vi "FuncVI-dtstr.vi"(5 "InstanceRef":T2, 9 "arg list":T1[](array[typedef]) {"num" format="%.2f"}) -> (0 "error out":bool, 3 "result":T1 {"num" format="%.2f"})   [LabVIEW 2021]
doc: "::: CalcExpress Toolkit :::\nCopyright (c) 2000-2026 Konstantin Shifershteyn. All rights reserved."
uses:
  cetypes.llb/CalcExpress Function Argument Info.ctl
  cetypes.llb/CalcExpress Instance RefNum.ctl
panel:
  in  "max arg num":i32=2
  in  "min arg num":i32
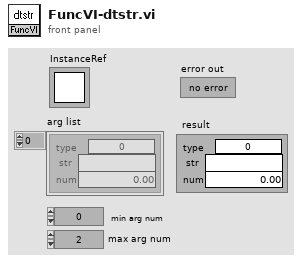
[diagram p1: front panel]
types:
  T1 = typedef "CalcExpress Function Argument Info.ctl" = cluster{"type":u32, "str":string, "num":dbl}
  T2 = typedef "CalcExpress Instance RefNum.ctl" = refnum<k1>
  T3 = cluster{"index":i32, "data type":enum32{"String", "DBL Number", "identifier", "1D Array of DBL", "2D Array of DBL", "CDB Number", "1D Array of CDB", "2D Array of CDB", "1D Array of String", "2D Array of String", "Unknown data type"}, "default num":dbl, "default str":string}
  T4 = cluster{"index":i32, "any type":i32, "default num":dbl, "default str":string}
  T5 = cluster{"index":i32, "any type":u32, "default num":dbl, "default str":string}[]
  T6 = enum32{"String", "DBL Number", "identifier", "1D Array of DBL", "2D Array of DBL", "CDB Number", "1D Array of CDB", "2D Array of CDB", "1D Array of String", "2D Array of String", "Unknown data type"}
  T7 = cluster{"data type":enum32{"String", "DBL Number", "identifier", "1D Array of DBL", "2D Array of DBL", "CDB Number", "1D Array of CDB", "2D Array of CDB", "1D Array of String", "2D Array of String", "Unknown data type"}, "data string":string, "num":dbl}
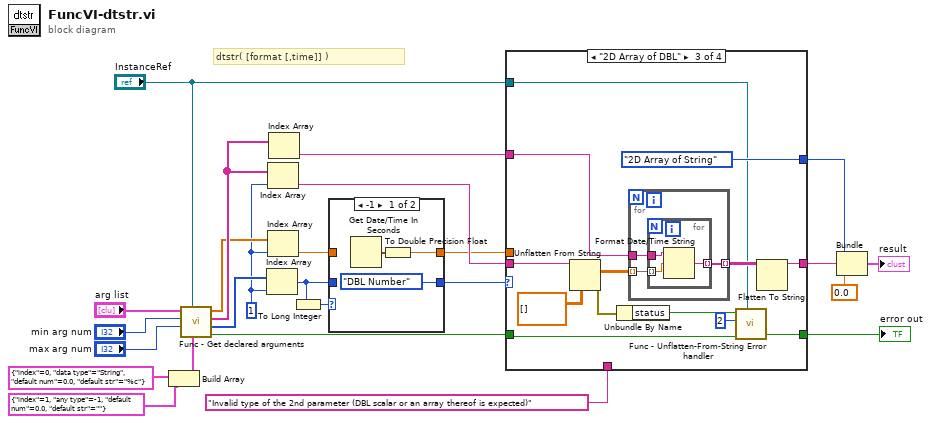
[diagram p0: block diagram]
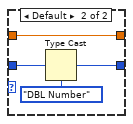
[diagram p2: hidden frame]
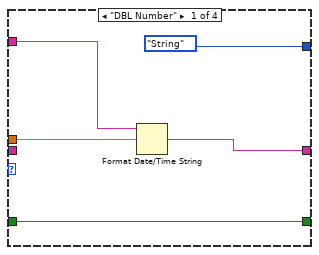
[diagram p3: hidden frame]
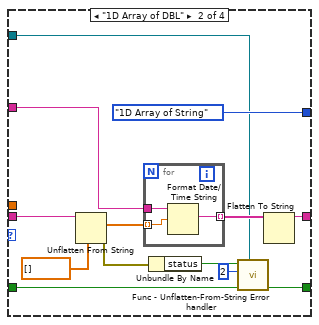
[diagram p4: hidden frame]
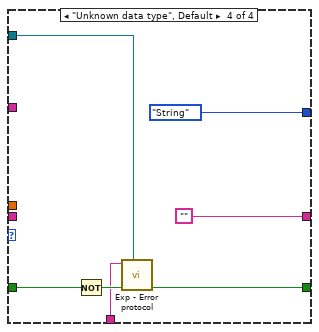
[diagram p5: hidden frame]
diagram:
  w6 = 1
  # "dtstr( [format [,time]] )"
  n1 = Build Array(T3 {"index"=0, "data type"=enum."String", "default num"=0.0, "default str"="%c"} ("arg descriptor"), T4 {"index"=1, "any type"=-1, "default num"=0.0, "default str"=""} ("arg descriptor")) -> (w23:T5)
  n2 = call "Func - Get declared arguments.vi"("arg descriptors"=w23, "InstanceRef"="InstanceRef", "max arg num"="max arg num", "min arg num"="min arg num", "arg list"="arg list") -> ("error out"=w19:bool, "type list"=w20:u32[], "str list"=w15:string[], "num list"=w14:dbl[])  [unwired: 3 in]
  n3 = Index Array(array=w20, index=w6) -> (element=w9:u32)
  n4 = Index Array(array=w15, index=w6) -> (element=w24:string)
  n5 = Index Array(array=w14, index=w6) -> (element=w7:dbl)
  n6 = Index Array(array=w15) -> (element=w21:string)  [unwired: 1 in]
  n7 = To Long Integer(number=w9) -> (32bit integer=w5:i32)
  n8 = case shown="-1" w5 {
    tunnel: [T6."DBL Number" ("data type") w30] -> w22
    tunnel: w9 -> [_ w31]
    tunnel: [w28 w32] -> w8
    tunnel: w7 -> [_ w32]
    frame -1 {
      n9 = Get Date/Time In Seconds() -> (seconds since 1Jan1904=w27:timestamp)
      n10 = To Double Precision Float(number=w27) -> (double precision float=w28:dbl)
    }
    frame Default {
      n11 = Type Cast(type=T6."DBL Number" ("data type"), x=w31) -> (*(type *) &x=w30:T6)
    }
  }
  n12 = case shown="\"2D Array of DBL\"" w22 {
    tunnel: w21 -> [w35 w44 w60 _]
    tunnel: [w33 w47 w63 ""] -> w13
    tunnel: w24 -> [_ w45 w61 _]
    tunnel: w8 -> [w34 _ _ _]
    tunnel: w19 -> [w37 w43 w57 w78]
    tunnel: [w37 w42 w58 w76] -> w18
    tunnel: "Invalid type of the 2nd parameter (DBL scalar or an array thereof is expected)" ("ErrStr") -> [_ _ _ w75]
    tunnel: "InstanceRef" -> [_ w41 w56 w74]
    tunnel: [T6."String" ("data type") T6."1D Array of String" ("data type") T6."2D Array of String" ("data type") T6."String" ("data type")] -> w11
    frame "DBL Number" {
      n13 = Format Date/Time String(time format string (%c)=w35, seconds (now)=w34) -> (date/time string=w33:string)  [unwired: 1 in]
    }
    frame "1D Array of DBL" {
      n14 = Unflatten From String(type=dbl[] [], binary string=w45) -> (value=w49:dbl[], error out=w38:errorcluster)  [unwired: 3 in, 1 out]
      n15 = for {
        tunnel: w49 -> [w53] mode=indexing
        tunnel: [w51] -> w48 mode=indexing
        tunnel: w44 -> [w52]
        n16 = Format Date/Time String(time format string (%c)=w52, seconds (now)=w53) -> (date/time string=w51:string)  [unwired: 1 in]
      }
      n17 = Unbundle By Name(w38) -> ("status"=w40:bool)
      n18 = call "Func - Unflatten-From-String Error handler.vi"("InstanceRef"=w41, "error in"=w43, "argument number"=2, "Unflatten Error status"=w40) -> ("error out"=w42:bool)  [unwired: 5 in]
      n19 = Flatten To String(anything=w48) -> (data string=w47:string)  [unwired: 3 in, 2 out]
    }
    frame "2D Array of DBL" {
      n20 = Unflatten From String(type=dbl[][] [], binary string=w61) -> (value=w65:dbl[][], error out=w54:errorcluster)  [unwired: 3 in, 1 out]
      n21 = Unbundle By Name(w54) -> ("status"=w55:bool)
      n22 = for {
        tunnel: w65 -> [w69] mode=indexing
        tunnel: [w68] -> w64 mode=indexing
        tunnel: w60 -> [w67]
        n23 = for {
          tunnel: w69 -> [w72] mode=indexing
          tunnel: [w70] -> w68 mode=indexing
          tunnel: w67 -> [w71]
          n24 = Format Date/Time String(time format string (%c)=w71, seconds (now)=w72) -> (date/time string=w70:string)  [unwired: 1 in]
        }
      }
      n25 = call "Func - Unflatten-From-String Error handler.vi"("InstanceRef"=w56, "error in"=w57, "argument number"=2, "Unflatten Error status"=w55) -> ("error out"=w58:bool)  [unwired: 5 in]
      n26 = Flatten To String(anything=w64) -> (data string=w63:string)  [unwired: 3 in, 2 out]
    }
    frame "Unknown data type", Default {
      n27 = Not(x=w78) -> (.not. x?=w77:bool)
      n28 = call "Exp - Error protocol.vi"("InstanceRef"=w74, "error in"=w77, "error message in"=w75) -> ("error out"=w76:bool)  [unwired: 5 in, 1 out]
    }
  }
  "error out" <- w18
  n29 = Bundle("data type"=w11, "data string"=w13, "num"=0.0) -> (→"result":T7)  [unwired: 1 in]
